vi "Read Width.vi"(8 "error in (no error)":errorcluster, 11 "Box in":refnum<class "Box.lvclass">) -> (0 "error out":errorcluster, 2 "Width":dbl, 3 "Box out":refnum<class "Box.lvclass">)   [LabVIEW 2026, in "Box.lvclass"]
doc: "Reads one field of this class's private data. Generated by lvai_create_accessors from the class private data control."
uses:
  Box.lvclass
  Box.lvclass/Box.ctl
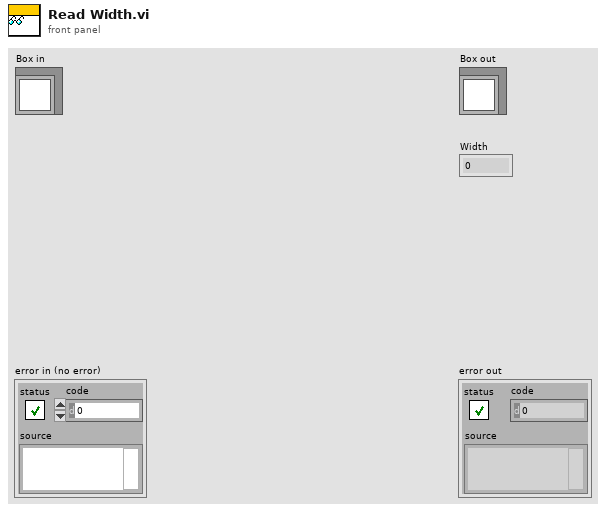
[diagram p1: front panel]
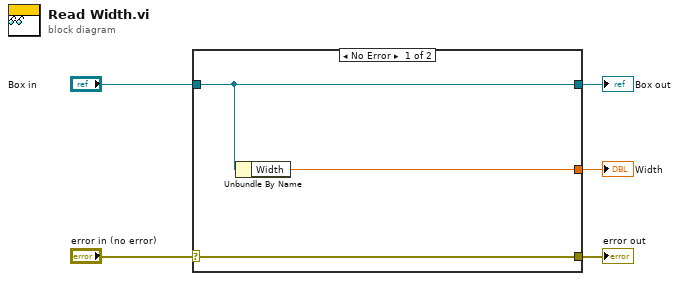
[diagram p0: block diagram]
diagram:
  n1 = case shown="No Error" "error in (no error)" {
    selector: "error in (no error)" -> [w8 w9]
    tunnel: [w8 w9] -> w4
    tunnel: [w7 w10] -> w2
    tunnel: "Box in" -> [w7 w10]
    tunnel: [w6 _] -> w1
    frame No Error {
      n2 = Unbundle By Name(w7) -> ("Width"=w6:dbl)
    }
    frame Error {
    }
  }
  "error out" <- w4
  "Box out" <- w2
  "Width" <- w1
